vi "Reflection Native Find Property.vi"(8 "error in (no error)":errorcluster, 10 "Property Name":string, 11 "Object Type in":refnum<k24>) -> (0 "error out":errorcluster, 2 "Property Info":refnum<k24>, 3 "Object Type out":refnum<k24>)   [LabVIEW 2026, in "ToastNotification.lvlib" / "Reflection DotNet.lvlib"]
doc: "Native System.Type.GetProperty call. Borrow Object Type in and acquire Property Info for Property Name. Object Type out aliases the input. Caller closes the acquired PropertyInfo; this VI does not read the property value or close the input Type."
uses:
  Reflection DotNet.lvlib
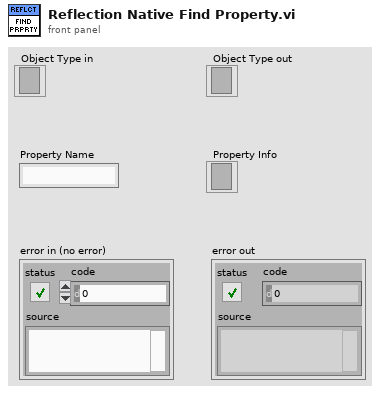
[diagram p1: front panel]
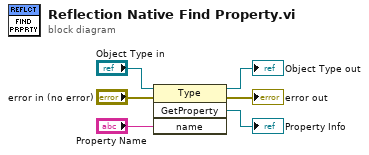
[diagram p0: block diagram]
diagram:
  n1 = invoke class="Type" method="GetProperty"(reference="Object Type in", error in="error in (no error)", "name"="Property Name") -> (reference out=→"Object Type out":refnum<k24>, error out=→"error out":errorcluster, "GetProperty"=→"Property Info":refnum<k24>)  [unwired: 1 in, 1 out]
